vi "FuncVI-vhQuery.vi"(5 "InstanceRef":T2, 9 "arg list":T1[](array[typedef]) {"num" format="%.2f"}) -> (0 "error out":bool, 3 "result":T1 {"num" format="%.2f"})   [LabVIEW 2021]
doc: "::: CalcExpress Toolkit :::\nCopyright (c) 2000-2026 Konstantin Shifershteyn. All rights reserved."
uses:
  cetypes.llb/CalcExpress Function Argument Info.ctl
  cetypes.llb/CalcExpress Instance RefNum.ctl
panel:
  in  "max arg num":i32=6
  in  "min arg num":i32=2
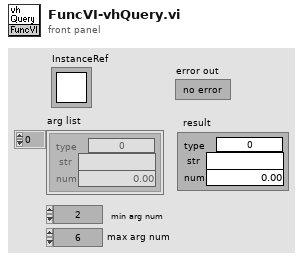
[diagram p1: front panel]
types:
  T1 = typedef "CalcExpress Function Argument Info.ctl" = cluster{"type":u32, "str":string, "num":dbl}
  T2 = typedef "CalcExpress Instance RefNum.ctl" = refnum<k1>
  T3 = enum32{"String", "DBL Number", "identifier", "1D Array of DBL", "2D Array of DBL", "CDB Number", "1D Array of CDB", "2D Array of CDB", "1D Array of String", "2D Array of String", "Unknown data type"}
  T4 = cluster{"index":i32, "data type":enum32{"String", "DBL Number", "identifier", "1D Array of DBL", "2D Array of DBL", "CDB Number", "1D Array of CDB", "2D Array of CDB", "1D Array of String", "2D Array of String", "Unknown data type"}, "default num":dbl, "default str":string}[]
  T5 = typedef "VarMan Variable Context Handle.ctl" = i32
  T6 = cluster{"data type":enum32{"String", "DBL Number", "identifier", "1D Array of DBL", "2D Array of DBL", "CDB Number", "1D Array of CDB", "2D Array of CDB", "1D Array of String", "2D Array of String", "Unknown data type"}, string, dbl}
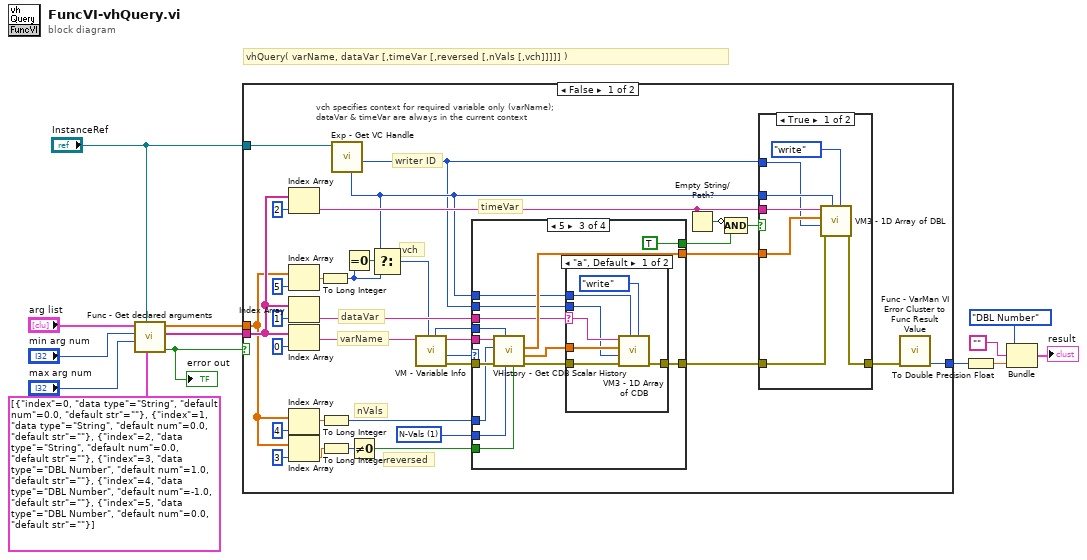
[diagram p0: block diagram]
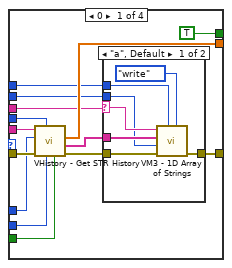
[diagram p3: hidden frame]
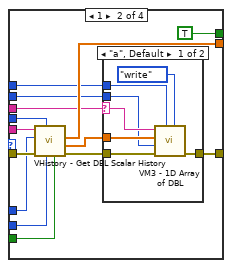
[diagram p5: hidden frame]
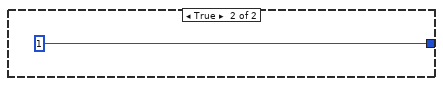
[diagram p9: hidden frame]
diagram:
  # "vhQuery( varName, dataVar [,timeVar [,reversed [,nVals [,vch]]]]] )"
  n1 = call "Func - Get declared arguments.vi"("arg descriptors"=T4 [{"index"=0, "data type"=enum."String", "default num"=0.0, "default str"=""}, {"index"=1, "data type"=enum."String", "default num"=0.0, "default str"=""}, {"index"=2, "data type"=enum."String", "default num"=0.0, "default str"=""}, {"index"=3, "data type"=enum."DBL Number", "default num"=1.0, "default str"=""}, {"index"=4, "data type"=enum."DBL Number", "default num"=-1.0, "default str"=""}, {"index"=5, "data type"=enum."DBL Number", "default num"=0.0, "default str"=""}], "InstanceRef"="InstanceRef", "max arg num"="max arg num", "min arg num"="min arg num", "arg list"="arg list") -> ("error out"=w12:bool, "str list"=w8:string[], "num list"=w2:dbl[])  [unwired: 3 in, 1 out]
  "error out" <- w12
  n2 = case shown="False" w12 {
    tunnel: w2 -> [w23 _]
    tunnel: w8 -> [w39 _]
    tunnel: [w14 1 ("code")] -> w1
    tunnel: "InstanceRef" -> [w21 _]
    frame False {
      w34 = u32 1 items=["TimeRange", "N-Vals", "NewVals"] ("mode")
      # "writer ID"
      # "nVals"
      # "reversed"
      # "vch"
      # "varName"
      # "timeVar"
      # "dataVar"
      # "vch specifies context for required variable only (varName);\ndataVar & timeVar are always in the current context"
      n3 = Index Array(array=w39, index=2) -> (element=w28:string)
      n4 = Index Array(array=w23, index=5) -> (element=w22:dbl)
      n5 = Index Array(array=w39, index=1) -> (element=w32:string)
      n6 = Index Array(array=w39, index=0) -> (element=w47:string)
      n7 = Index Array(array=w23, index=4) -> (element=w36:dbl)
      n8 = Index Array(array=w23, index=3) -> (element=w38:dbl)
      n9 = To Long Integer(number=w22) -> (32bit integer=w19:i32)
      n10 = To Long Integer(number=w36) -> (32bit integer=w33:i32)
      n11 = To Long Integer(number=w38) -> (32bit integer=w37:i32)
      n12 = call "Exp - Get VC Handle.vi"("InstanceRef"=w21) -> ("writer ID"=w16:u32, "VC Handle"=w17:T5)  [unwired: 5 in, 2 out]
      n13 = Equal To 0?(x=w19) -> (x = 0?=w20:bool)
      n14 = Not Equal To 0?(x=w37) -> (x != 0?=w35:bool)
      n15 = Select(t=w17, s=w20, f=w19) -> (s? t:f=w18:T5)
      n16 = call "VM - Variable Info.vi"("VC Handle"=w18, "name_spec"=w47) -> ("error out"=w25:errorcluster, "var type"=w46:u32, "var name"=w45:string, "var VC Handle"=w44:T5)  [unwired: 4 in, 2 out]
      n17 = case shown="5" w46 {
        tunnel: w45 -> [w70 w92 w114 _]
        tunnel: w44 -> [w61 w83 w105 _]
        tunnel: w35 -> [w69 w91 w113 _]
        tunnel: w34 -> [w68 w90 w112 _]
        tunnel: w25 -> [w67 w89 w111 w123]
        tunnel: w33 -> [w66 w88 w110 _]
        tunnel: [w65 w87 w109 _] -> w27
        tunnel: w32 -> [w64 w86 w108 _]
        tunnel: w17 -> [w60 w82 w104 _]
        tunnel: [w59 w81 w103 w123] -> w26
        tunnel: [TRUE TRUE TRUE _] -> w30
        tunnel: w16 -> [w57 w79 w101 _]
        frame 0 {
          n18 = call "VHistory - Get STR History.vi"("reverse order (T)"=w69, "mode"=w68, "VC Handle"=w61, "error in"=w67, "N vals (all)"=w66, "name_spec"=w70) -> ("error out"=w62:errorcluster, "history"=w63:string[], "time stamps"=w65:dbl[])  [unwired: 1 in, 2 out]
          n19 = case shown="\"a\", Default" w64 {
            selector: w64 -> [w77 _]
            tunnel: w63 -> [w76 _]
            tunnel: w62 -> [w75 w78]
            tunnel: [w74 w78] -> w59
            tunnel: w60 -> [w73 _]
            tunnel: w57 -> [w71 _]
            frame "a", Default {
              n20 = call "VM3 - 1D Array of Strings.vi"("cmd (read)"=enum16{"create", "destroy", "write", "read"}."write", "VC Handle"=w73, "error in"=w75, "writer ID"=w71, "value in"=w76, "name_spec"=w77) -> ("error out"=w74:errorcluster)  [unwired: 2 in, 3 out]
            }
            frame "" {
            }
          }
        }
        frame 1 {
          n21 = call "VHistory - Get DBL Scalar History.vi"("reverse order (T)"=w91, "mode"=w90, "VC Handle"=w83, "error in"=w89, "N vals (all)"=w88, "name_spec"=w92) -> ("error out"=w84:errorcluster, "history"=w85:dbl[], "time stamps"=w87:dbl[])  [unwired: 1 in, 2 out]
          n22 = case shown="\"a\", Default" w86 {
            selector: w86 -> [w99 _]
            tunnel: w85 -> [w98 _]
            tunnel: w84 -> [w97 w100]
            tunnel: [w96 w100] -> w81
            tunnel: w82 -> [w95 _]
            tunnel: w79 -> [w93 _]
            frame "a", Default {
              n23 = call "VM3 - 1D Array of DBL.vi"("cmd (read)"=enum16{"create", "destroy", "write", "read"}."write", "VC Handle"=w95, "error in"=w97, "writer ID"=w93, "value in"=w98, "name_spec"=w99) -> ("error out"=w96:errorcluster)  [unwired: 2 in, 3 out]
            }
            frame "" {
            }
          }
        }
        frame 5 {
          n24 = call "VHistory - Get CDB Scalar History.vi"("reverse order (T)"=w113, "mode"=w112, "VC Handle"=w105, "error in"=w111, "N vals (all)"=w110, "name_spec"=w114) -> ("error out"=w106:errorcluster, "history"=w107:cdb[], "time stamps"=w109:dbl[])  [unwired: 1 in, 2 out]
          n25 = case shown="\"a\", Default" w108 {
            selector: w108 -> [w121 _]
            tunnel: w107 -> [w120 _]
            tunnel: w106 -> [w119 w122]
            tunnel: [w118 w122] -> w103
            tunnel: w104 -> [w117 _]
            tunnel: w101 -> [w115 _]
            frame "a", Default {
              n26 = call "VM3 - 1D Array of CDB.vi"("cmd (read)"=enum16{"create", "destroy", "write", "read"}."write", "VC Handle"=w117, "error in"=w119, "writer ID"=w115, "value in"=w120, "name_spec"=w121) -> ("error out"=w118:errorcluster)  [unwired: 2 in, 3 out]
            }
            frame "" {
            }
          }
        }
        frame 2, Default {
        }
      }
      n27 = Empty String/Path?(string/path=w28) -> (empty?=w31:bool)
      n28 = Compound Arithmetic op=AND(invert w31, w30) -> (w29:bool)
      n29 = case shown="True" w29 {
        tunnel: w26 -> [w55 w56]
        tunnel: [w54 w56] -> w15
        tunnel: w17 -> [w53 _]
        tunnel: w28 -> [w52 _]
        tunnel: w27 -> [w51 _]
        tunnel: w16 -> [w49 _]
        frame True {
          n30 = call "VM3 - 1D Array of DBL.vi"("cmd (read)"=enum16{"create", "destroy", "write", "read"}."write", "VC Handle"=w53, "error in"=w55, "writer ID"=w49, "value in"=w51, "name_spec"=w52) -> ("error out"=w54:errorcluster)  [unwired: 2 in, 3 out]
        }
        frame False {
        }
      }
      n31 = call "Func - VarMan VI Error Cluster to Func Result Value.vi"("VarMan VI error in"=w15) -> ("CE Function Result Value"=w14:i32)  [unwired: 10 in]
    }
    frame True {
    }
  }
  n32 = To Double Precision Float(number=w1) -> (double precision float=w7:dbl)
  n33 = Bundle("data type"=T3."DBL Number", "", w7) -> (→"result":T6)  [unwired: 1 in]
